vi "Acquire Tag Heading.vi"(8 "error in (no error)":errorcluster, 9 "Command Info In":T1) -> (0 "error out":errorcluster, 1 "Command Info Out":T1, 2 "Acquired":bool, 3 "Target Heading":dbl)   [LabVIEW 2025]
doc: "Stop, then wait up to 1 second for a new Limelight 3a heartbeat with tv=1 and tid>=1. Target yaw = Pigeon yaw - tx for a forward-facing camera. Camera table is limelight. Pipeline must already be AprilTag. No fresh tag means Acquired=false."
uses:
  <vilib>/Rock Robotics/WPI/Framework/Command Status Info.ctl
  <vilib>/Rock Robotics/WPI/Framework/Completion Status.ctl
  <vilib>/Rock Robotics/WPI/Framework/Completion Notifier.ctl
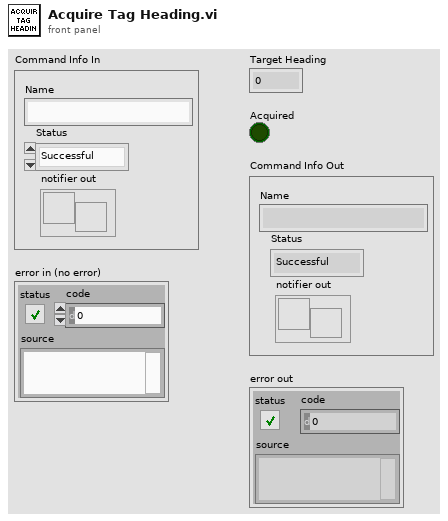
[diagram p1: front panel]
types:
  T1 = typedef "Command Status Info.ctl" = cluster{"Name":string, "Status":T2, "notifier out":T3}
  T2 = typedef "Completion Status.ctl" = enum16{"Successful", "Aborted", "Incomplete"}
  T3 = typedef "Completion Notifier.ctl" = refnum<notifier>
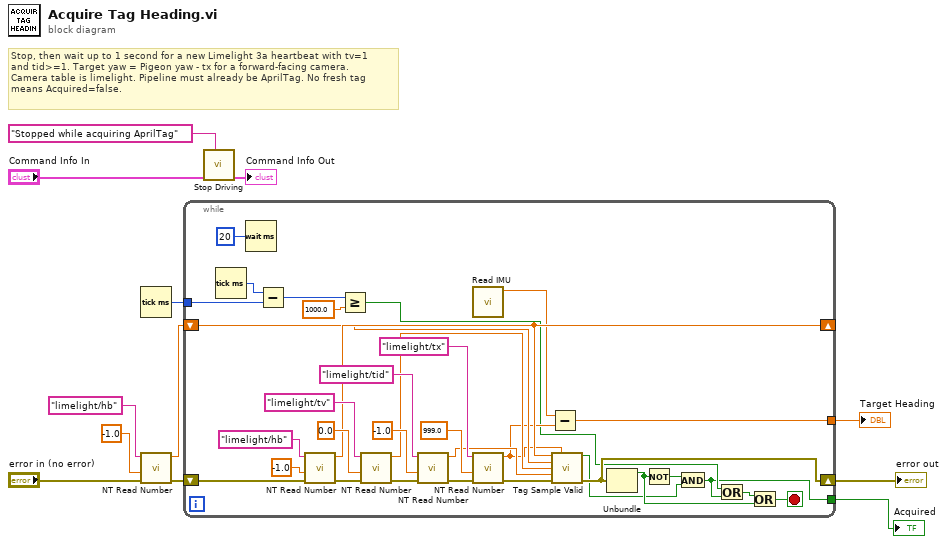
[diagram p0: block diagram]
diagram:
  # "Stop, then wait up to 1 second for a new Limelight 3a heartbeat with tv=1\nand tid>=1. Target yaw = Pigeon yaw - tx for a forward-facing camera.\nCamera table is limelight. Pipeline must already be AprilTag. No fresh tag\nmeans Acquired=false."
  n1 = Tick Count (ms)() -> (millisecond timer value=w6:u32)
  n2 = call <vilib>:"NT Read Number.vi"("error in"="error in (no error)", "default value"=-1.0, "name"="limelight/hb") -> ("error out"=w7:errorcluster, "value"=w8:dbl)  [unwired: 6 in, 1 out]
  n3 = while {
    shift-right: [w35] -> _
    shift-left: w8 -> [w34]
    shift-right: [w32] -> w1
    shift-left: w7 -> [w33]
    tunnel: w6 -> [w27]
    tunnel: [w14] -> w3
    tunnel: [w13] -> w2
    stop <- w16 stop-if-true
    n4 = Tick Count (ms)() -> (millisecond timer value=w28:u32)
    n5 = Wait (ms)(milliseconds to wait=u32 20) -> ()  [unwired: 1 out]
    n6 = Subtract(x=w28, y=w27) -> (x-y=w26:u32)
    n7 = call <vilib>:"NT Read Number.vi"("error in"=w33, "default value"=-1.0, "name"="limelight/hb") -> ("error out"=w23:errorcluster, "value"=w35:dbl)  [unwired: 6 in, 1 out]
    n8 = Greater Or Equal?(x=w26, y=1000.0) -> (x >= y?=w25:bool)
    n9 = call <vilib>:"NT Read Number.vi"("error in"=w23, "default value"=0.0, "name"="limelight/tv") -> ("error out"=w22:errorcluster, "value"=w31:dbl)  [unwired: 6 in, 1 out]
    n10 = call <vilib>:"NT Read Number.vi"("error in"=w22, "default value"=-1.0, "name"="limelight/tid") -> ("error out"=w21:errorcluster, "value"=w30:dbl)  [unwired: 6 in, 1 out]
    n11 = call "Read IMU.vi"() -> ("Heading"=w24:dbl)  [unwired: 11 in]
    n12 = call <vilib>:"NT Read Number.vi"("error in"=w21, "default value"=999.0, "name"="limelight/tx") -> ("error out"=w15:errorcluster, "value"=w29:dbl)  [unwired: 6 in, 1 out]
    n13 = Subtract(x=w24, y=w29) -> (x-y=w14:dbl)
    n14 = call "Tag Sample Valid.vi"("Heartbeat"=w35, "tx Degrees"=w29, "Previous Heartbeat"=w34, "Target Valid"=w31, "Tag ID"=w30, "error in (no error)"=w15) -> ("Valid Sample"=w18:bool, "error out"=w32:errorcluster)  [unwired: 8 in]
    n15 = Unbundle(w32) -> ("status"=w20:bool)  [unwired: 2 out]
    n16 = Not(x=w20) -> (.not. x?=w19:bool)
    n17 = And(x=w19, y=w18) -> (x .and. y?=w13:bool)
    n18 = Or(x=w25, y=w13) -> (x .or. y?=w17:bool)
    n19 = Or(x=w17, y=w20) -> (x .or. y?=w16:bool)
  }
  "Target Heading" <- w3
  "Acquired" <- w2
  "error out" <- w1
  n20 = call "Stop Driving.vi"("Description"="Stopped while acquiring AprilTag", "Command Info In"="Command Info In") -> ("Command Info Out"=→"Command Info Out":T1)  [unwired: 9 in]
